vi "lire fichier rapport.vi"(1 "Nom du régulateur":string, 2 "Fichier de rapport":path) -> (0 "début du profil":timestamp)   [LabVIEW 2022 SP3]
uses:
  Enum/Enum 1.ctl
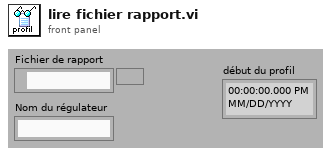
[diagram p1: front panel]
types:
  T1 = typedef "Enum 1.ctl" = enum16{"ouverture fichier profil", "régulateur conserné", "extrait date et heure", "date et heure actuelles"}
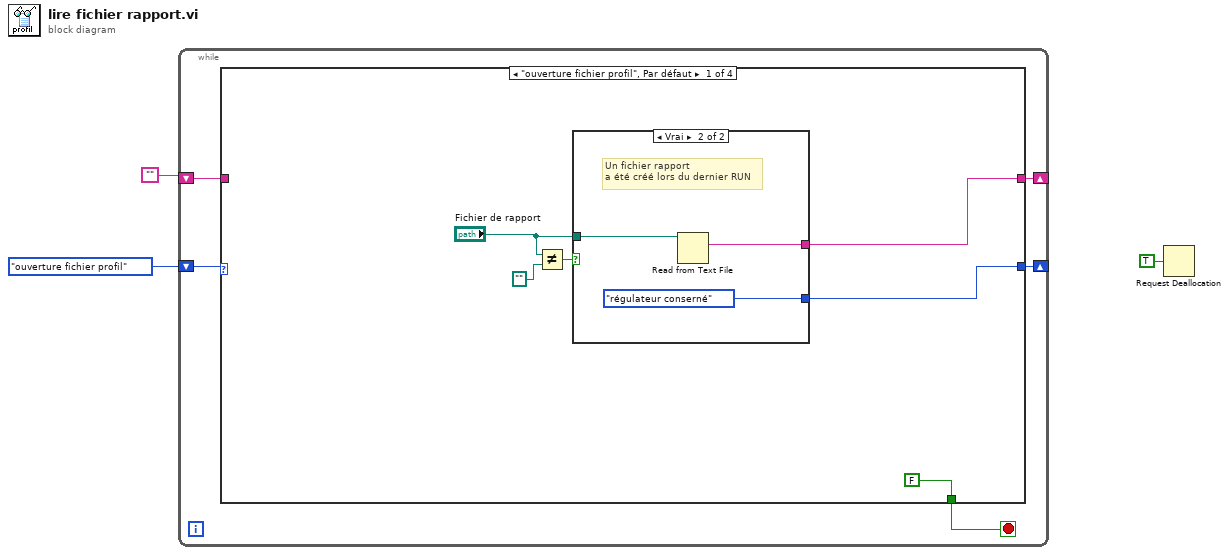
[diagram p0: block diagram]
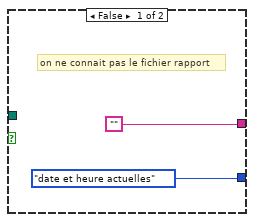
[diagram p2: hidden frame]
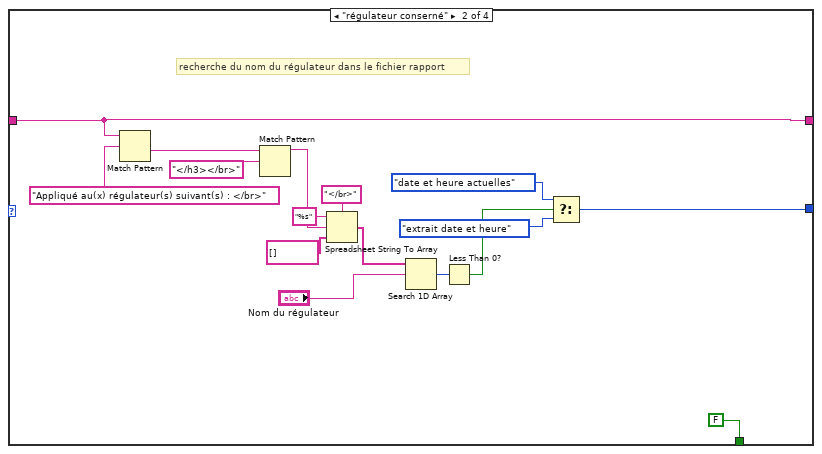
[diagram p3: hidden frame]
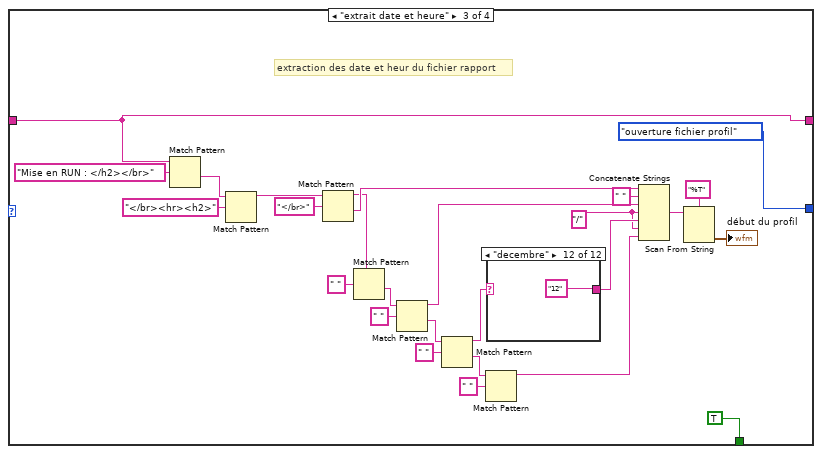
[diagram p4: hidden frame]
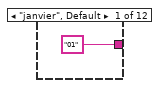
[diagram p5: hidden frame]
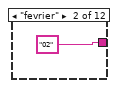
[diagram p6: hidden frame]
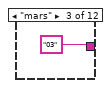
[diagram p7: hidden frame]
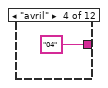
[diagram p8: hidden frame]
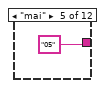
[diagram p9: hidden frame]
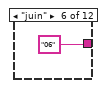
[diagram p10: hidden frame]
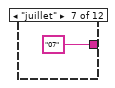
[diagram p11: hidden frame]
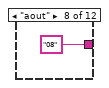
[diagram p12: hidden frame]
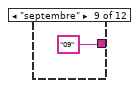
[diagram p13: hidden frame]
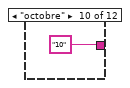
[diagram p14: hidden frame]
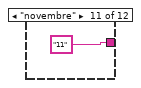
[diagram p15: hidden frame]
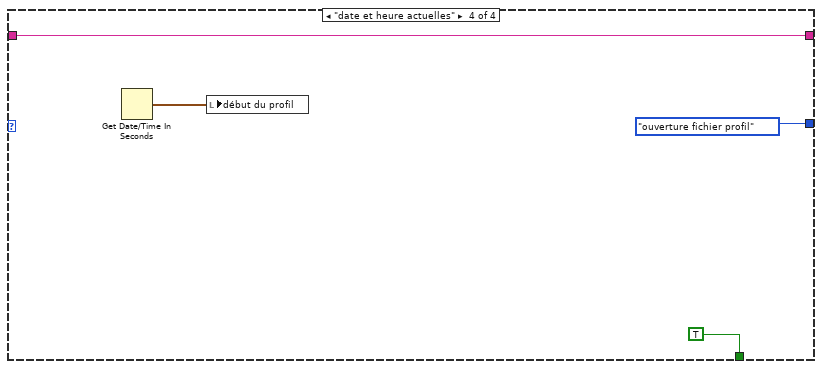
[diagram p16: hidden frame]
diagram:
  n1 = while {
    shift-right: [w6] -> _
    shift-left: Enum_1."ouverture fichier profil" ("Énum") -> [w8]
    shift-right: [w7] -> _
    shift-left: "" -> [w5]
    stop <- w4 stop-if-true
    n2 = case shown="\"ouverture fichier profil\", Par défaut" w8 {
      tunnel: [w11 w20 w36 w74] -> w7
      tunnel: [w10 w22 Enum_1."ouverture fichier profil" ("Énum") Enum_1."ouverture fichier profil" ("Énum")] -> w6
      tunnel: w5 -> [_ w20 w36 w74]
      tunnel: [FALSE FALSE TRUE TRUE] -> w4
      frame "ouverture fichier profil", Default {
        n3 = Not Equal?(x="Fichier de rapport", y=path "") -> (x != y?=w12:bool)
        n4 = case shown="Vrai" w12 {
          tunnel: "Fichier de rapport" -> [_ w19]
          tunnel: ["" w18] -> w11
          tunnel: [Enum_1."date et heure actuelles" ("Énum") Enum_1."régulateur conserné" ("Énum")] -> w10
          frame False {
            # "on ne connait pas le fichier rapport"
          }
          frame True {
            # "Un fichier rapport \na été créé lors du dernier RUN"
            n5 = Read from Text File(file (use dialog)=w19) -> (text=w18:string)  [unwired: 3 in, 3 out]
          }
        }
      }
      frame "régulateur conserné" {
        # "recherche du nom du régulateur dans le fichier rapport"
        n6 = Match Pattern(string=w20, regular expression="Appliqué au(x) régulateur(s) suivant(s) : </br>" ("expression régulière")) -> (after substring=w27:string)  [unwired: 1 in, 3 out]
        n7 = Match Pattern(string=w27, regular expression="</h3></br>" ("expression régulière")) -> (before substring=w26:string)  [unwired: 1 in, 3 out]
        n8 = Spreadsheet String To Array(delimiter (Tab)="</br>" ("séparateur (Tabulation)"), format string="%s" ("chaîne de format"), spreadsheet string=w26, array type (2D Dbl)=string[] [] ("type de tableau (2D de dbl)")) -> (array=w33:string[])
        n9 = Search 1D Array(1D array=w33, element="Nom du régulateur") -> (index of element=w35:i32)  [unwired: 1 in]
        n10 = Less Than 0?(x=w35) -> (x < 0?=w25:bool)
        n11 = Select(t=Enum_1."date et heure actuelles" ("Énum"), s=w25, f=Enum_1."extrait date et heure" ("Énum")) -> (s? t:f=w22:T1)
      }
      frame "extrait date et heure" {
        w55 = "/" ("chaîne")
        # "extraction des date et heur du fichier rapport"
        n12 = Match Pattern(string=w36, regular expression="Mise en RUN : </h2></br>" ("expression régulière")) -> (after substring=w41:string)  [unwired: 1 in, 3 out]
        n13 = Match Pattern(string=w41, regular expression="</br><hr><h2>" ("expression régulière")) -> (before substring=w58:string)  [unwired: 1 in, 3 out]
        n14 = Match Pattern(string=w58, regular expression="</br>" ("expression régulière")) -> (before substring=w45:string, after substring=w60:string)  [unwired: 1 in, 2 out]
        n15 = Match Pattern(string=w45, regular expression=" " ("expression régulière")) -> (after substring=w48:string)  [unwired: 1 in, 3 out]
        n16 = Match Pattern(string=w48, regular expression=" " ("expression régulière")) -> (before substring=w49:string, after substring=w50:string)  [unwired: 1 in, 2 out]
        n17 = Match Pattern(string=w50, regular expression=" " ("expression régulière")) -> (before substring=w56:string, after substring=w53:string)  [unwired: 1 in, 2 out]
        n18 = Match Pattern(string=w53, regular expression=" " ("expression régulière")) -> (before substring=w54:string)  [unwired: 1 in, 3 out]
        n19 = case shown="\"decembre\"" w56 {
          tunnel: ["01" "02" "03" "04" "05" "06" "07" "08" "09" "10" "11" "12"] -> w57
          frame "janvier", Default {
          }
          frame "fevrier" {
          }
          frame "mars" {
          }
          frame "avril" {
          }
          frame "mai" {
          }
          frame "juin" {
          }
          frame "juillet" {
          }
          frame "aout" {
          }
          frame "septembre" {
          }
          frame "octobre" {
          }
          frame "novembre" {
          }
          frame "decembre" {
          }
        }
        n20 = Concatenate Strings(w60, " " ("chaîne"), w49, w55, w57, w55, w54) -> (w59:string)
        n21 = Scan From String(format string="%T" ("chaîne de format"), input string=w59) -> (output 1=→"début du profil":timestamp)  [unwired: 3 in, 3 out]
      }
      frame "date et heure actuelles" {
        n22 = Get Date/Time In Seconds() -> (seconds since 1Jan1904=w77:timestamp)
        n23 = local write "début du profil"(w77) -> ()
      }
    }
  }
  n24 = Request Deallocation(TRUE ("flag")) -> ()
